vi "RemoteVI Cancel Popups.vi"(0 "hWnd":u64, 5 "posts":cluster{"msg":u32, "wParam":u64, "lParam":i64}[](array[cluster]), 11 "error in":errorcluster) -> (15 "error out":errorcluster)   [LabVIEW 2020, in "RemoteVI.lvlib"]
doc: "For a click OUTSIDE every popup: a button-down sends WM_CANCELMODE to hWnd with user32 SendMessageTimeoutW, which closes every open LabVIEW popup (a sent WM_CANCELMODE closes the whole menu, submenus included, measured); any other message (the matching button-up) does nothing. Nothing is posted. No VI Server call."
uses:
  RemoteVI.lvlib
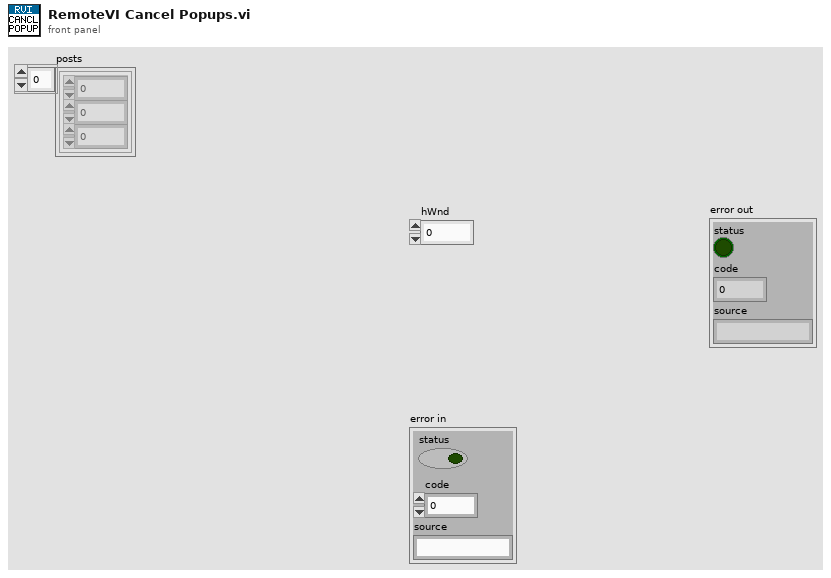
[diagram p1: front panel]
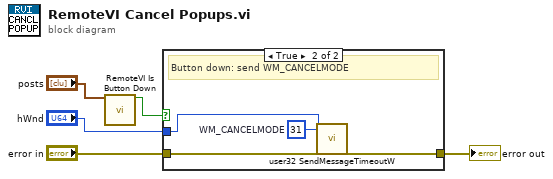
[diagram p0: block diagram]
diagram:
  n1 = call "RemoteVI Is Button Down.vi"("posts"="posts") -> ("button down?"=w4:bool)  [unwired: 14 in]
  n2 = case shown="True" w4 {
    tunnel: "error in" -> [w6 w7]
    tunnel: "hWnd" -> [_ w8]
    tunnel: [w6 w10] -> w5
    frame False {
    }
    frame True {
      w9 = u32 31  # WM_CANCELMODE
      # "Button down: send WM_CANCELMODE"
      n3 = call "user32 SendMessageTimeoutW.vi"("hWnd"=w8, "Msg"=w9, "error in"=w7) -> ("error out"=w10:errorcluster)  [unwired: 22 in, 2 out]
    }
  }
  "error out" <- w5
